vi "FuncVI-viState.vi"(5 "InstanceRef":T2, 9 "arg list":T1[](array[typedef]) {"num" format="%.2f"}) -> (0 "error out":bool, 3 "result":T1 {"num" format="%.2f"})   [LabVIEW 2021]
doc: "::: CalcExpress Toolkit :::\nCopyright (c) 2000-2026 Konstantin Shifershteyn. All rights reserved."
uses:
  cetypes.llb/CalcExpress Function Argument Info.ctl
  cetypes.llb/CalcExpress Instance RefNum.ctl
panel:
  in  "max arg num":i32=2
  in  "min arg num":i32=1
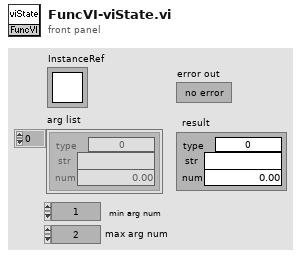
[diagram p1: front panel]
types:
  T1 = typedef "CalcExpress Function Argument Info.ctl" = cluster{"type":u32, "str":string, "num":dbl}
  T2 = typedef "CalcExpress Instance RefNum.ctl" = refnum<k1>
  T3 = enum32{"String", "DBL Number", "identifier", "1D Array of DBL", "2D Array of DBL", "CDB Number", "1D Array of CDB", "2D Array of CDB", "1D Array of String", "2D Array of String", "Unknown data type"}
  T4 = cluster{"index":i32, "data type":enum32{"String", "DBL Number", "identifier", "1D Array of DBL", "2D Array of DBL", "CDB Number", "1D Array of CDB", "2D Array of CDB", "1D Array of String", "2D Array of String", "Unknown data type"}, "default num":dbl, "default str":string}[]
  T5 = enum32{"Bad", "Idle", "Run top level", "Running"}
  T6 = enum32{"Invalid", "Standard", "Closed", "Hidden", "Minimized", "Maximized"}
  T7 = cluster{"use this constant to specify a predefined type":enum32{"String", "DBL Number", "identifier", "1D Array of DBL", "2D Array of DBL", "CDB Number", "1D Array of CDB", "2D Array of CDB", "1D Array of String", "2D Array of String", "Unknown data type"}, string, "code":dbl}
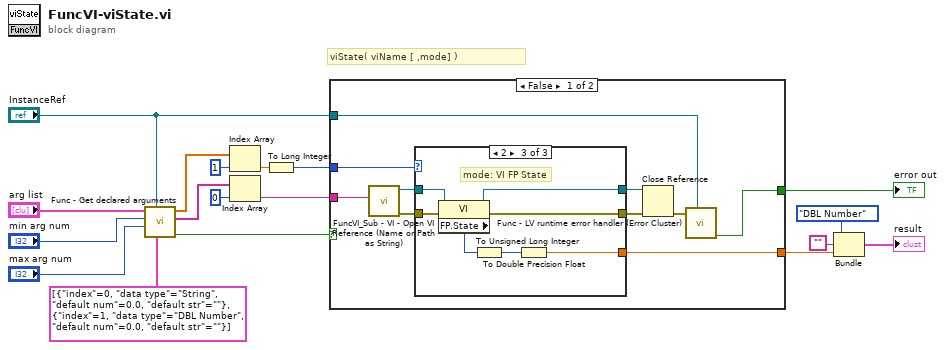
[diagram p0: block diagram]
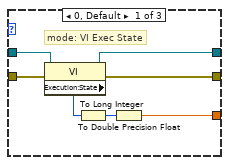
[diagram p2: hidden frame]
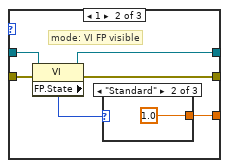
[diagram p3: hidden frame]
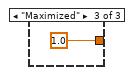
[diagram p5: hidden frame]
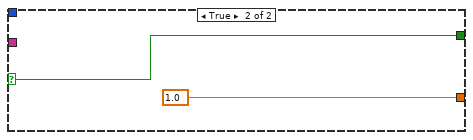
[diagram p6: hidden frame]
diagram:
  # "viState( viName [ ,mode] )"
  n1 = call "Func - Get declared arguments.vi"("arg descriptors"=T4 [{"index"=0, "data type"=enum."String", "default num"=0.0, "default str"=""}, {"index"=1, "data type"=enum."DBL Number", "default num"=0.0, "default str"=""}] ("args descriptors"), "InstanceRef"="InstanceRef", "max arg num"="max arg num", "min arg num"="min arg num", "arg list"="arg list") -> ("error out"=w4:bool, "str list"=w11:string[], "num list"=w12:dbl[])  [unwired: 3 in, 1 out]
  n2 = Index Array(array=w12, index=1) -> (element=w10:dbl)
  n3 = Index Array(array=w11, index=0) -> (element=w2:string)
  n4 = To Long Integer(number=w10) -> (32bit integer=w1:i32)
  n5 = case shown="False" w4 {
    selector: w4 -> [_ w52]
    tunnel: w2 -> [w28 _]
    tunnel: [w20 w52] -> w8
    tunnel: "InstanceRef" -> [w21 _]
    tunnel: [w23 1.0 ("code")] -> w3
    tunnel: w1 -> [w19 _]
    frame False {
      n6 = call "FuncVI_Sub - VI - Open VI Reference (Name or Path as String).vi"("VI name or path"=w28) -> ("error out"=w27:errorcluster, "VI Refnum"=w26:refnum<vi>)  [unwired: 9 in]
      n7 = case shown="2" w19 {
        tunnel: w27 -> [w35 w40 w49]
        tunnel: w26 -> [w34 w41 w50]
        tunnel: [w33 w39 w48] -> w24
        tunnel: [w32 w38 w47] -> w25
        tunnel: [w29 w36 w44] -> w23
        frame 0, Default {
          # "mode: VI Exec State"
          n8 = property class="VI"(reference=w34, error in=w35) -> (reference out=w33:refnum<vi>, error out=w32:errorcluster, "Execution:State"=w31:T5)
          n9 = To Long Integer(number=w31) -> (32bit integer=w30:i32)
          n10 = To Double Precision Float(number=w30) -> (double precision float=w29:dbl)
        }
        frame 1 {
          # "mode: VI FP visible"
          n11 = property class="VI"(reference=w41, error in=w40) -> (reference out=w39:refnum<vi>, error out=w38:errorcluster, "FP.State"=w37:T6)
          n12 = case shown="\"Standard\"" w37 {
            tunnel: [_ 1.0 1.0] -> w36
            frame Default {
            }
            frame "Standard" {
            }
            frame "Maximized" {
            }
          }
        }
        frame 2 {
          # "mode: VI FP State"
          n13 = property class="VI"(reference=w50, error in=w49) -> (reference out=w48:refnum<vi>, error out=w47:errorcluster, "FP.State"=w46:T6)
          n14 = To Unsigned Long Integer(number=w46) -> (unsigned 32bit integer=w45:u32)
          n15 = To Double Precision Float(number=w45) -> (double precision float=w44:dbl)
        }
      }
      n16 = Close Reference(reference=w24, error in (no error)=w25) -> (error out=w22:errorcluster)
      n17 = call "Func - LV runtime error handler (Error Cluster).vi"("InstanceRef"=w21, "LabVIEW error"=w22) -> ("error out"=w20:bool)  [unwired: 4 in, 3 out]
    }
    frame True {
    }
  }
  "error out" <- w8
  n18 = Bundle("use this constant to specify a predefined type"=T3."DBL Number", "", "code"=w3) -> (→"result":T7)  [unwired: 1 in]
